vi "Plugin_Manager.vi"(8 "error in (no error)":errorcluster={"status"=FALSE, "code"=0, "source"="\"\""}, 10 "requests":string="START_REQ", 11 "Plugin manifests":string="MANIFEST_JSON") -> (0 "error out":errorcluster={"status"=FALSE, "code"=0, "source"="\"\""}, 2 "status ok":bool, 3 "Plugin status/events":string)   [LabVIEW 2026]
doc: "INTENT: Central plugin executive validating manifests, starting instances, and dispatching worker results."
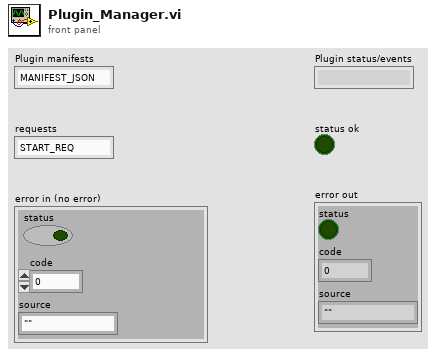
[diagram p1: front panel]
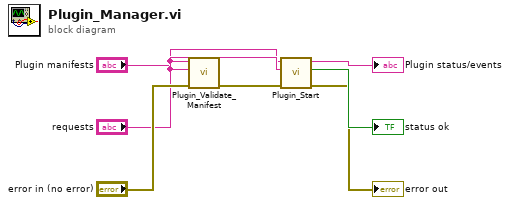
[diagram p0: block diagram]
diagram:
  n1 = call "Plugin_Validate_Manifest.vi"("error in (no error)"="error in (no error)", "target capability"="requests", "PluginManifest"="Plugin manifests") -> ("error out"=w4:errorcluster)  [unwired: 6 in, 2 out]
  n2 = call "Plugin_Start.vi"("error in (no error)"=w4, "typed args"="requests", "Plugin ID"="Plugin manifests") -> ("error out"=→"error out":errorcluster, "status ok"=→"status ok":bool, "Instance ID"=→"Plugin status/events":string)  [unwired: 6 in]
